vi "test panel for 2nd.vi"(8 "error in":errorcluster caption="エラー入力（エラーなし）", 11 "S New Info and MiN":T2={"Sample Sequence"="GATGATGATGATGATGAT", "Right Read MIN"=6, "Filter P"=0, "STD Type"=enum."Region", "Base Table"=[], "Selection"=enum."10kHz", "noise MAX"=3, "Sample name"=""} {"Base Table"."Value 3" format="%.2g"}) -> (0 "error out":errorcluster caption="エラー出力", 1 "SB_ANA":T1, 3 "S New Info and MiN out":T2={"Sample Sequence"="GATGATGATGATGATGAT", "Right Read MIN"=6, "Filter P"=0, "STD Type"=enum."Region", "Base Table"=[], "Selection"=enum."10kHz", "noise MAX"=3, "Sample name"=""} {"Base Table"."Value 3" format="%.2g"})   [LabVIEW 2018]
panel:
  out "element":string
  in  "Sequence 手入力":bool
  in  "Right Read#":bool
  in  "Sequence Set":bool
  in  "Set":bool
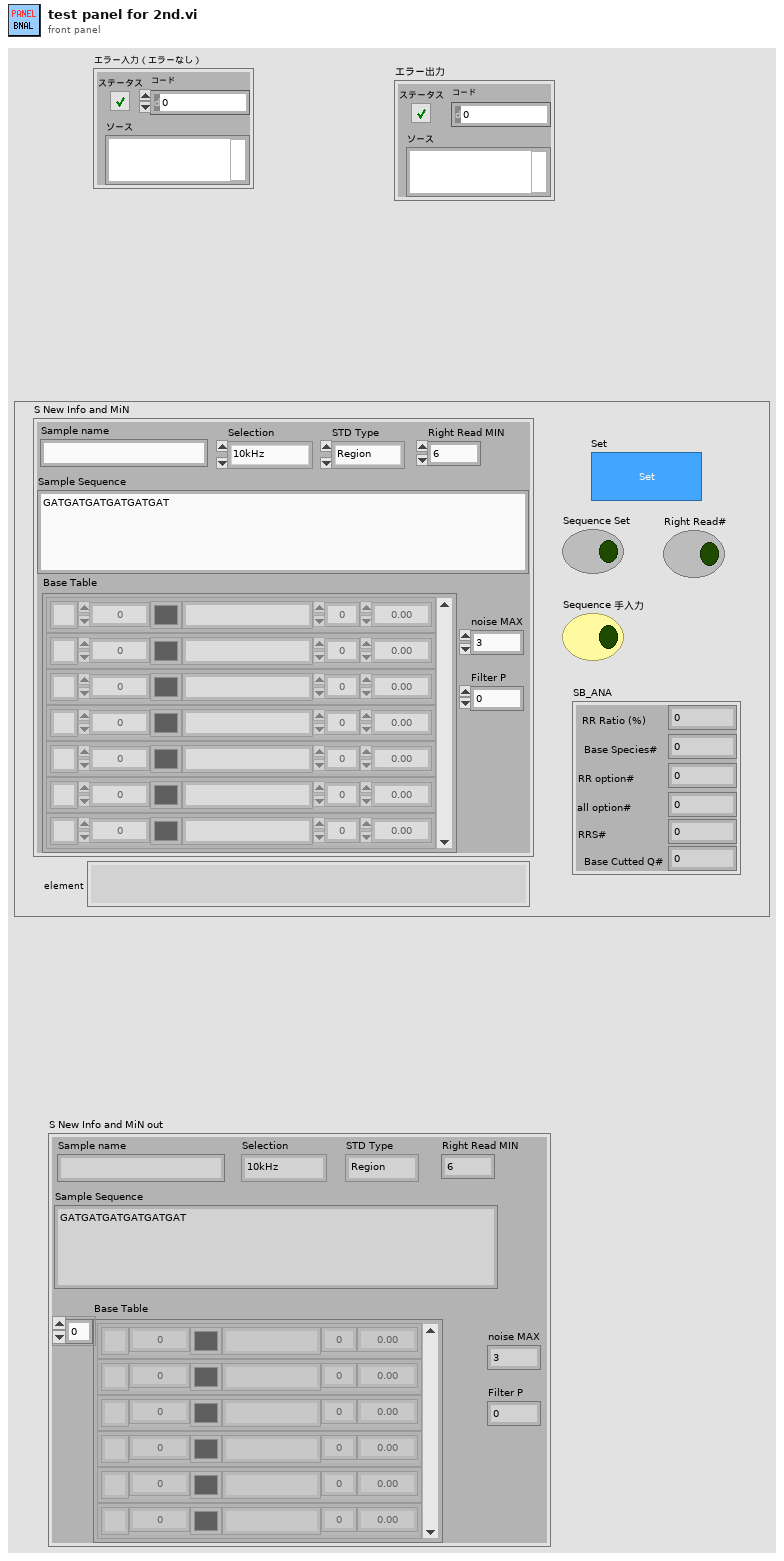
[diagram p1: front panel]
types:
  T1 = cluster{"RR Ratio (%)":dbl, "Base Species#":i32, "RR option#":i32, "all option#":i32, "RRS#":i32, "Base Cutted Q#":i32}
  T2 = cluster{"Sample Sequence":string, "Right Read MIN":i32, "Filter P":i32, "STD Type":enum16{"Region", "Each", "Fixed"}, "Base Table":cluster{"Name":string, "Value":dbl, "Color":u32, "Name 2":string, "Value 2":dbl, "Value 3":dbl}[], "Selection":enum16{"10kHz", "100kHz"}, "noise MAX":i32, "Sample name":string}
  T3 = cluster{"Name":string, "Value":dbl, "Color":u32, "Name 2":string, "Value 2":dbl, "Value 3":dbl}[]
  T4 = cluster{"Sample Sequence":string, "Right Read MIN out":i32, "Filter P":i32, "STD Type":enum16{"Region", "Each", "Fixed"}, "Base Table":cluster{"Name":string, "Value":dbl, "Color":u32, "Name 2":string, "Value 2":dbl, "Value 3":dbl}[], "Selection":enum16{"10kHz", "100kHz"}, "noise MAX":i32, "Sample name":string}
  T5 = cluster{"Sample Sequence":string, "Right Read MIN":i32, "Filter P":i32, "STD Type":enum16{"Region", "Each", "Fixed"}, "Base All Composition":cluster{"Name":string, "Value":dbl, "Color":u32, "Name 2":string, "Value 2":dbl, "Value 3":dbl}[], "Selection":enum16{"10kHz", "100kHz"}, "noise MAX":i32, "Sample name":string}
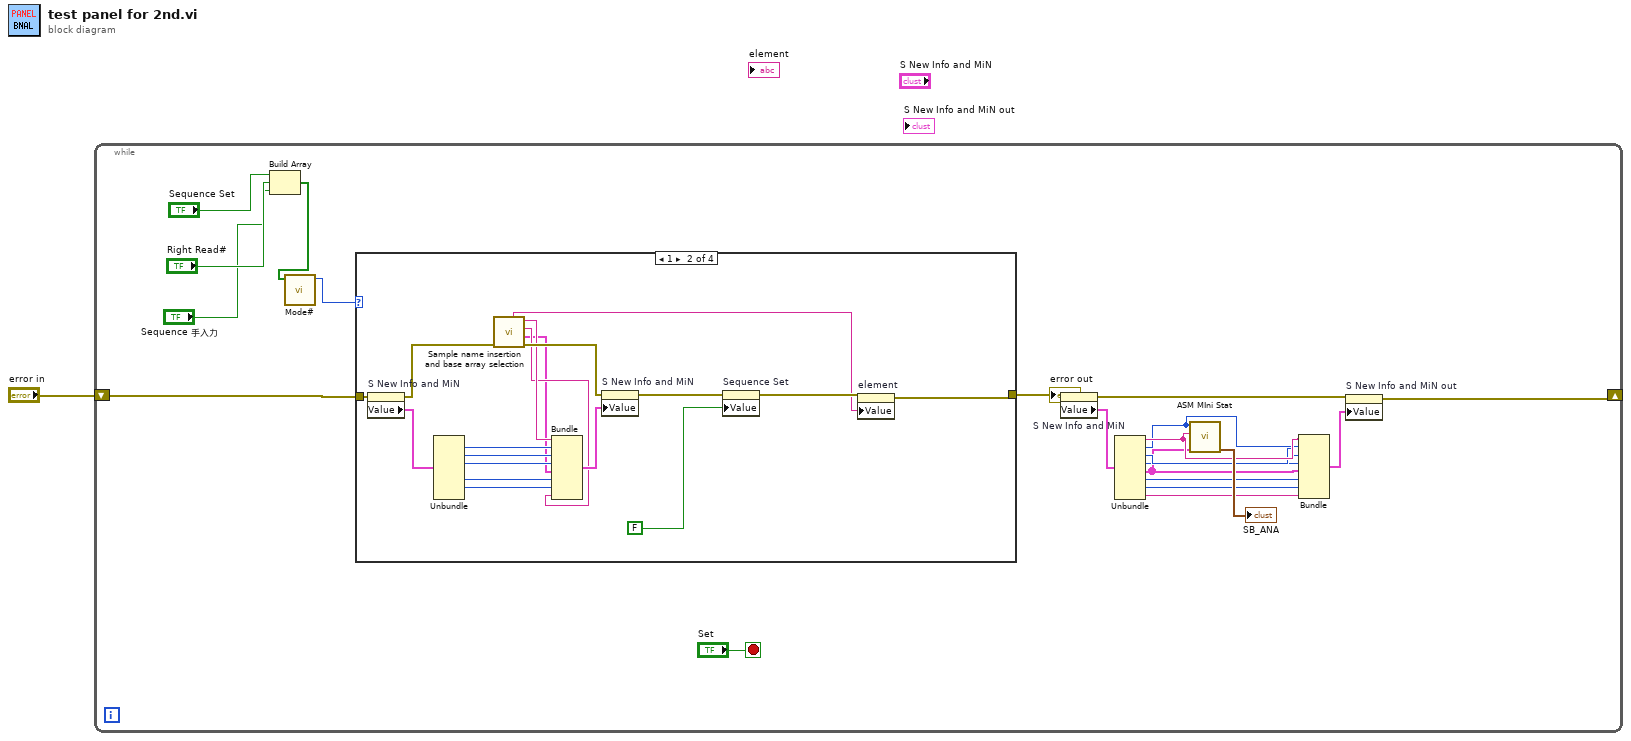
[diagram p0: block diagram]
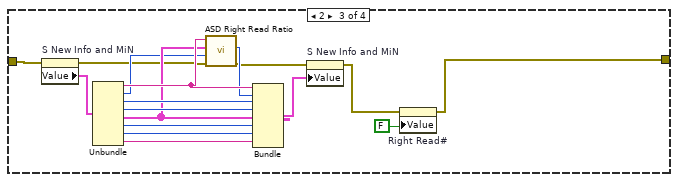
[diagram p3: hidden frame]
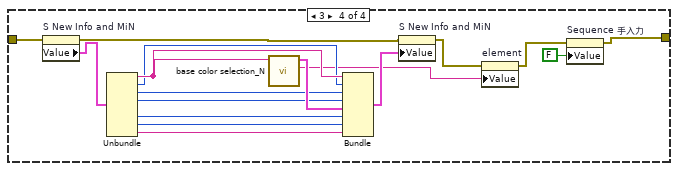
[diagram p4: hidden frame]
diagram:
  n1 = while {
    shift-right: [w2] -> _
    shift-left: "error in" -> [w22]
    stop <- "Set" stop-if-true
    n2 = Build Array("Sequence Set", "Right Read#", "Sequence 手入力") -> (w20:bool[])
    n3 = call "Mode#.vi"("MR all data"=w20) -> ("Mode#"=w17:i32)  [unwired: 10 in]
    n4 = case shown="1" w17 {
      tunnel: w22 -> [w23 w41 w58 w66]
      tunnel: [w23 w25 w47 w65] -> w14
      frame 0, Default {
      }
      frame 1 {
        n5 = property on="S New Info and MiN" class="Clust (strict)"(error in=w41) -> (error out=w31:errorcluster, "Value"=w40:T2)  [unwired: 1 in, 1 out]
        n6 = Unbundle(w40) -> ("Right Read MIN"=w38:i32, "Filter P"=w37:i32, "STD Type"=w36:enum16{"Region", "Each", "Fixed"}, "Selection"=w35:enum16{"10kHz", "100kHz"}, "noise MAX"=w34:i32)  [unwired: 3 out]
        n7 = call "Sample name insertion and base array selection.vi"("error in"=w31) -> ("error out"=w30:errorcluster, "Base Table"=w27:T3, "Sample name"=w28:string, "Sample Sequence"=w29:string, "element"=w24:string)  [unwired: 6 in]
        n8 = Bundle("Sample Sequence"=w29, "Right Read MIN"=w38, "Filter P"=w37, "STD Type"=w36, "Base Table"=w27, "Selection"=w35, "noise MAX"=w34, "Sample name"=w28) -> (w39:T2)  [unwired: 1 in]
        n9 = property on="S New Info and MiN" class="Clust (strict)"(error in=w30, "Value"=w39) -> (error out=w33:errorcluster)  [unwired: 1 in, 1 out]
        n10 = property on="Sequence Set" class="Bool (strict)"(error in=w33, "Value"=FALSE ("配列選択入力")) -> (error out=w26:errorcluster)  [unwired: 1 in, 1 out]
        n11 = property on="element" class="Str"(error in=w26, "Value"=w24) -> (error out=w25:errorcluster)  [unwired: 1 in, 1 out]
      }
      frame 2 {
        n12 = property on="S New Info and MiN" class="Clust (strict)"(error in=w58) -> (error out=w43:errorcluster, "Value"=w57:T2)  [unwired: 1 in, 1 out]
        n13 = Unbundle(w57) -> ("Sample Sequence"=w55:string, "Right Read MIN"=w45:i32, "Filter P"=w54:i32, "STD Type"=w53:enum16{"Region", "Each", "Fixed"}, "Base Table"=w52:T3, "Selection"=w51:enum16{"10kHz", "100kHz"}, "noise MAX"=w50:i32, "Sample name"=w49:string)
        n14 = call "ASD Right Read Ratio.vi"("error in"=w43, "Right Read MIN"=w45, "Base Table"=w52, "Sample Sequence"=w55) -> ("error out"=w42:errorcluster, "Right Read MIN out"=w44:i32)  [unwired: 4 in, 2 out]
        n15 = Bundle("Sample Sequence"=w55, "Right Read MIN out"=w44, "Filter P"=w54, "STD Type"=w53, "Base Table"=w52, "Selection"=w51, "noise MAX"=w50, "Sample name"=w49) -> (w56:T4)  [unwired: 1 in]
        n16 = property on="S New Info and MiN" class="Clust (strict)"(error in=w42, "Value"=w56) -> (error out=w48:errorcluster)  [unwired: 1 in, 1 out]
        n17 = property on="Right Read#" class="Bool (strict)"(error in=w48, "Value"=FALSE ("Right Read#")) -> (error out=w47:errorcluster)  [unwired: 1 in, 1 out]
      }
      frame 3 {
        n18 = property on="S New Info and MiN" class="Clust (strict)"(error in=w66) -> (error out=w62:errorcluster, "Value"=w67:T2)  [unwired: 1 in, 1 out]
        n19 = Unbundle(w67) -> ("Sample Sequence"=w75:string, "Right Read MIN"=w68:i32, "Filter P"=w69:i32, "STD Type"=w70:enum16{"Region", "Each", "Fixed"}, "Selection"=w71:enum16{"10kHz", "100kHz"}, "noise MAX"=w72:i32, "Sample name"=w73:string)  [unwired: 1 out]
        n20 = call "base color selection_N.vi"("Sample Sequence"=w75) -> ("element"=w61:string, "Base All Composition"=w74:T3)  [unwired: 9 in]
        n21 = Bundle("Sample Sequence"=w75, "Right Read MIN"=w68, "Filter P"=w69, "STD Type"=w70, "Base All Composition"=w74, "Selection"=w71, "noise MAX"=w72, "Sample name"=w73) -> (w63:T5)  [unwired: 1 in]
        n22 = property on="S New Info and MiN" class="Clust (strict)"(error in=w62, "Value"=w63) -> (error out=w60:errorcluster)  [unwired: 1 in, 1 out]
        n23 = property on="element" class="Str"(error in=w60, "Value"=w61) -> (error out=w59:errorcluster)  [unwired: 1 in, 1 out]
        n24 = property on="Sequence 手入力" class="Bool (strict)"(error in=w59, "Value"=FALSE ("Sequence 手入力")) -> (error out=w65:errorcluster)  [unwired: 1 in, 1 out]
      }
    }
    n25 = property on="S New Info and MiN" class="Clust (strict)"(error in=w14) -> (error out=w12:errorcluster, "Value"=w13:T2)  [unwired: 1 in, 1 out]
    n26 = Unbundle(w13) -> ("Sample Sequence"=w10:string, "Right Read MIN"=w9:i32, "Filter P"=w8:i32, "STD Type"=w7:enum16{"Region", "Each", "Fixed"}, "Base Table"=w6:T3, "Selection"=w5:enum16{"10kHz", "100kHz"}, "noise MAX"=w4:i32, "Sample name"=w3:string)
    n27 = call "ASM MIni Stat.vi"("Base Table"=w6, "Sample Sequence"=w10, "Right Read MIN"=w9) -> ("SB_ANA"=→"SB_ANA":T1)  [unwired: 6 in, 2 out]
    n28 = Bundle("Sample Sequence"=w10, "Right Read MIN"=w9, "Filter P"=w8, "STD Type"=w7, "Base Table"=w6, "Selection"=w5, "noise MAX"=w4, "Sample name"=w3) -> (w11:T2)  [unwired: 1 in]
    n29 = property on="S New Info and MiN out" class="Clust (strict)"(error in=w12, "Value"=w11) -> (error out=w2:errorcluster)  [unwired: 1 in, 1 out]
  }
